vi "Truncate String Core.vi"(8 "Error In":errorcluster, 9 "Max Length (32)":i32=32, 10 "Connector (...)":string="...", 11 "String in":string) -> (0 "Error Out":errorcluster, 1 "length out":i32, 2 "length in":i32, 3 "String out":string)   [LabVIEW 2021, in "Strings.lvlib"]
uses:
  Strings.lvlib
panel:
  # "see the License on the block diagram (Ctrl+E or Window:Show Block Diagram)"
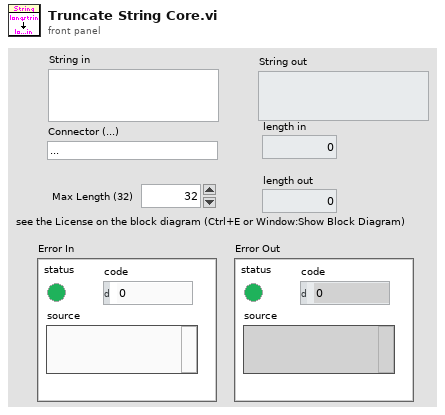
[diagram p1: front panel]
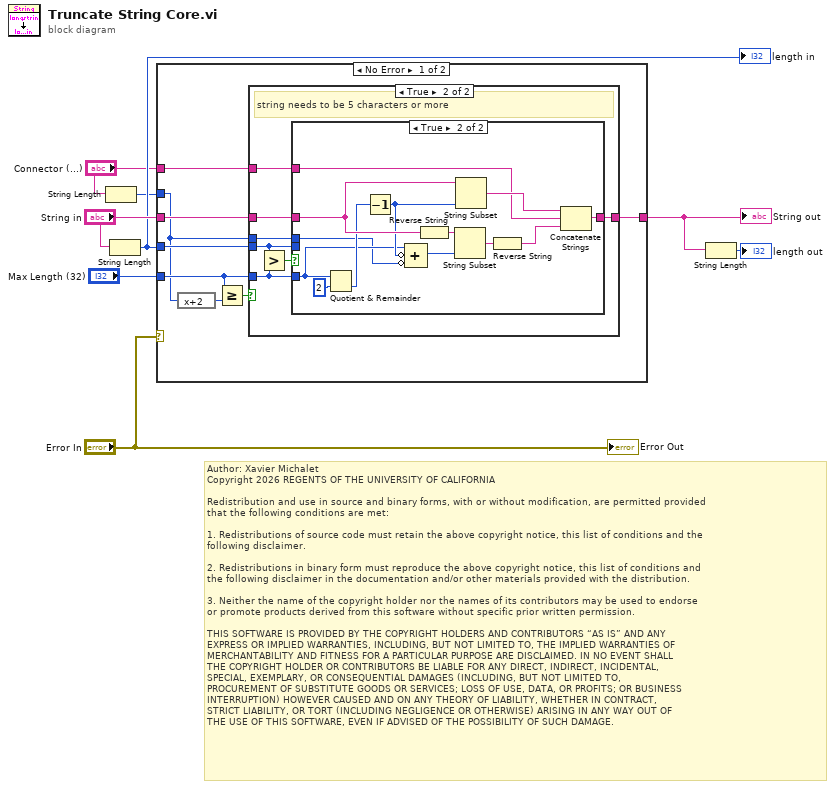
[diagram p0: block diagram]
diagram:
  # "Author: Xavier Michalet\nCopyright 2026 REGENTS OF THE UNIVERSITY OF CALIFORNIA\n\nRedistribution and use in source and binary forms, with or without modification, are permitted provided\nthat the following conditions are met:\n\n1. Redistributions of source code must retain the above copyright notice, this list of conditions and the\nfollowing disclaimer.\n\n2. Redistributions in binary form must reproduce the above copyright notice, this list of conditions and\nthe following disclaimer in the documentation and/or other materials provided with the distribution.\n\n3. Neither the name of the copyright holder nor the names of its contributors may be used to endorse \nor promote products derived from this software without specific prior written permission.\n\nTHIS SOFTWARE IS PROVIDED BY THE COPYRIGHT HOLDERS AND CONTRIBUTORS “AS IS” AND ANY \nEXPRESS OR IMPLIED WARRANTIES, INCLUDING, BUT NOT LIMITED TO, THE IMPLIED WARRANTIES OF\nMERCHANTABILITY AND FITNESS FOR A PARTICULAR PURPOSE ARE DISCLAIMED. IN NO EVENT SHALL\nTHE COPYRIGHT HOLDER OR CONTRIBUTORS BE LIABLE FOR ANY DIRECT, INDIRECT, INCIDENTAL, \nSPECIAL, EXEMPLARY, OR CONSEQUENTIAL DAMAGES (INCLUDING, BUT NOT LIMITED TO, \nPROCUREMENT OF SUBSTITUTE GOODS OR SERVICES; LOSS OF USE, DATA, OR PROFITS; OR BUSINESS\nINTERRUPTION) HOWEVER CAUSED AND ON ANY THEORY OF LIABILITY, WHETHER IN CONTRACT, \nSTRICT LIABILITY, OR TORT (INCLUDING NEGLIGENCE OR OTHERWISE) ARISING IN ANY WAY OUT OF\nTHE USE OF THIS SOFTWARE, EVEN IF ADVISED OF THE POSSIBILITY OF SUCH DAMAGE."
  n1 = String Length(string="Connector (...)") -> (length=w1:i32)
  n2 = String Length(string="String in") -> (length=w5:i32)
  "length in" <- w5
  n3 = case shown="No Error" "Error In" {
    tunnel: "String in" -> [w16 w39]
    tunnel: [w15 w39] -> w7
    tunnel: w5 -> [w14 _]
    tunnel: "Max Length (32)" -> [w13 _]
    tunnel: "Connector (...)" -> [w11 _]
    tunnel: w1 -> [w9 _]
    frame No Error {
      n4 = expression code="x+2"(w9) -> (w10:i32)
      n5 = Greater Or Equal?(x=w13, y=w10) -> (x >= y?=w12:bool)
      n6 = case shown="True" w12 {
        tunnel: w16 -> [w17 w24]
        tunnel: [w17 w22] -> w15
        tunnel: w14 -> [_ w21]
        tunnel: w13 -> [_ w20]
        tunnel: w11 -> [_ w19]
        tunnel: w9 -> [_ w18]
        frame False {
        }
        frame True {
          # "string needs to be 5 characters or more"
          n7 = Greater?(x=w21, y=w20) -> (0:w23:bool)
          n8 = case shown="True" w23 {
            tunnel: w24 -> [w25 w37]
            tunnel: [w25 w32] -> w22
            tunnel: w21 -> [_ _]
            tunnel: w20 -> [_ w28]
            tunnel: w19 -> [_ w27]
            tunnel: w18 -> [_ w26]
            frame False {
              # "no need to truncate"
            }
            frame True {
              n9 = Quotient & Remainder(x=w28, y=2) -> (floor(x/y)=w29:i32)  [unwired: 1 out]
              n10 = Decrement(x=w29) -> (x-1=w30:i32)
              n11 = Compound Arithmetic op=ADD(w28, invert w30, invert w26) -> (w31:i32)
              n12 = Reverse String(1:w37) -> (0:w36:string)
              n13 = String Subset(string=w36, length (rest)=w31) -> (substring=w35:string)  [unwired: 1 in]
              n14 = String Subset(string=w37, length (rest)=w30) -> (substring=w34:string)  [unwired: 1 in]
              n15 = Reverse String(1:w35) -> (0:w33:string)
              n16 = Concatenate Strings(w34, w27, w33) -> (w32:string)
            }
          }
        }
      }
    }
    frame Error {
    }
  }
  "String out" <- w7
  n17 = String Length(string=w7) -> (length=→"length out":i32)
  "Error Out" <- "Error In"
